vi "Write Report Path.vi"(10 "Report Path":path, 11 "Test Report.Template in":refnum<class "Test Report.Template.lvclass">) -> (3 "Test Report.Template out":refnum<class "Test Report.Template.lvclass">)   [LabVIEW 2020, in "Caraya.lvlib" / "Test Report.Template.lvclass"]
uses:
  Test Report.Template.lvclass
  Test Report.Template.lvclass/Test Report.Template.ctl
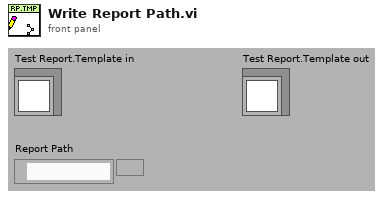
[diagram p1: front panel]
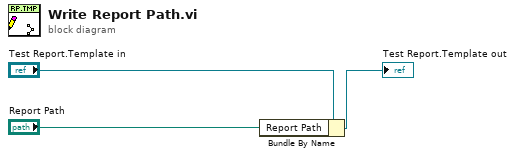
[diagram p0: block diagram]
diagram:
  n1 = Bundle By Name(cluster="Test Report.Template in", "Report Path"="Report Path") -> (→"Test Report.Template out":refnum<class "Test Report.Template.lvclass">)
